vi "Save Profi map Pressure.vi"(0 "Pressure":T2(array[cluster]), 1 "configuration file path":path, 3 "error in":errorcluster, 4 "Write":bool) -> (7 "Array":T2(array[cluster]), 10 "error out":errorcluster)   [LabVIEW 2025]
uses:
  <vilib>/Utility/config.llb/NI_LVConfig.lvlib
  controls/Tempratures.ctl
  controls/Profi address.ctl
  <vilib>/Utility/config.llb/Read Key (String).vi
  <vilib>/Utility/config.llb/Write Key (String).vi
  controls/Power Meters.ctl
panel:
  in  "Power Meters":cluster{"Select Item 3":T1, "Combo Box 2":T3}[](array[cluster])
  in  "Tempratures":cluster{"Sensor":T4, "Profi":T1}[][](array[cluster])
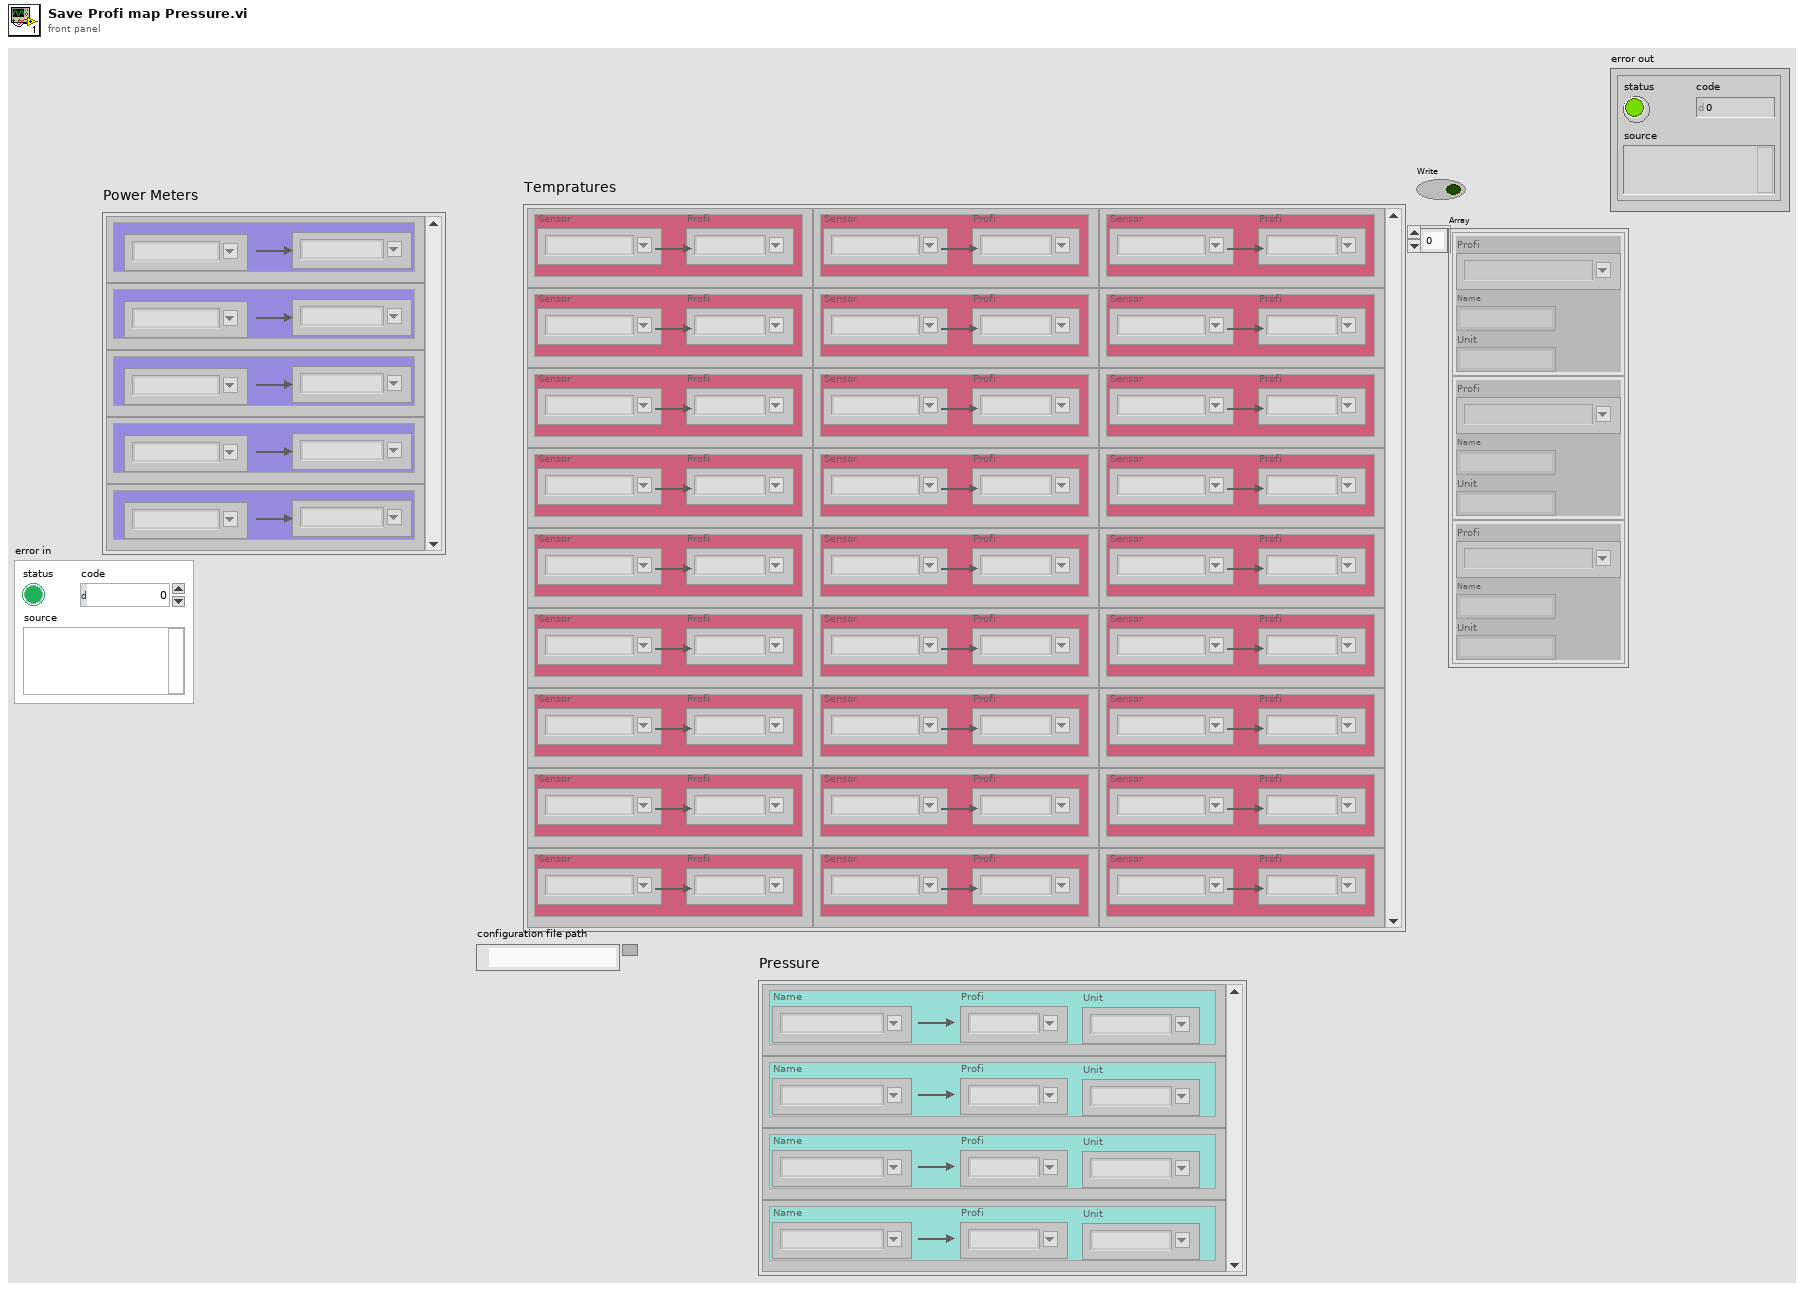
[diagram p1: front panel]
types:
  T1 = typedef "Profi address.ctl" = string
  T2 = cluster{"Profi":T1, "Name":string, "Unit":string}[]
  T3 = typedef "Power Meters.ctl" = string
  T4 = typedef "Tempratures.ctl" = string
  T5 = cluster{"Profi":T1, "Name":string, "Unit":string}
  T6 = typedef "NI_LVConfig.lvlib/Config Data RefNum.ctl" = refnum<k1>
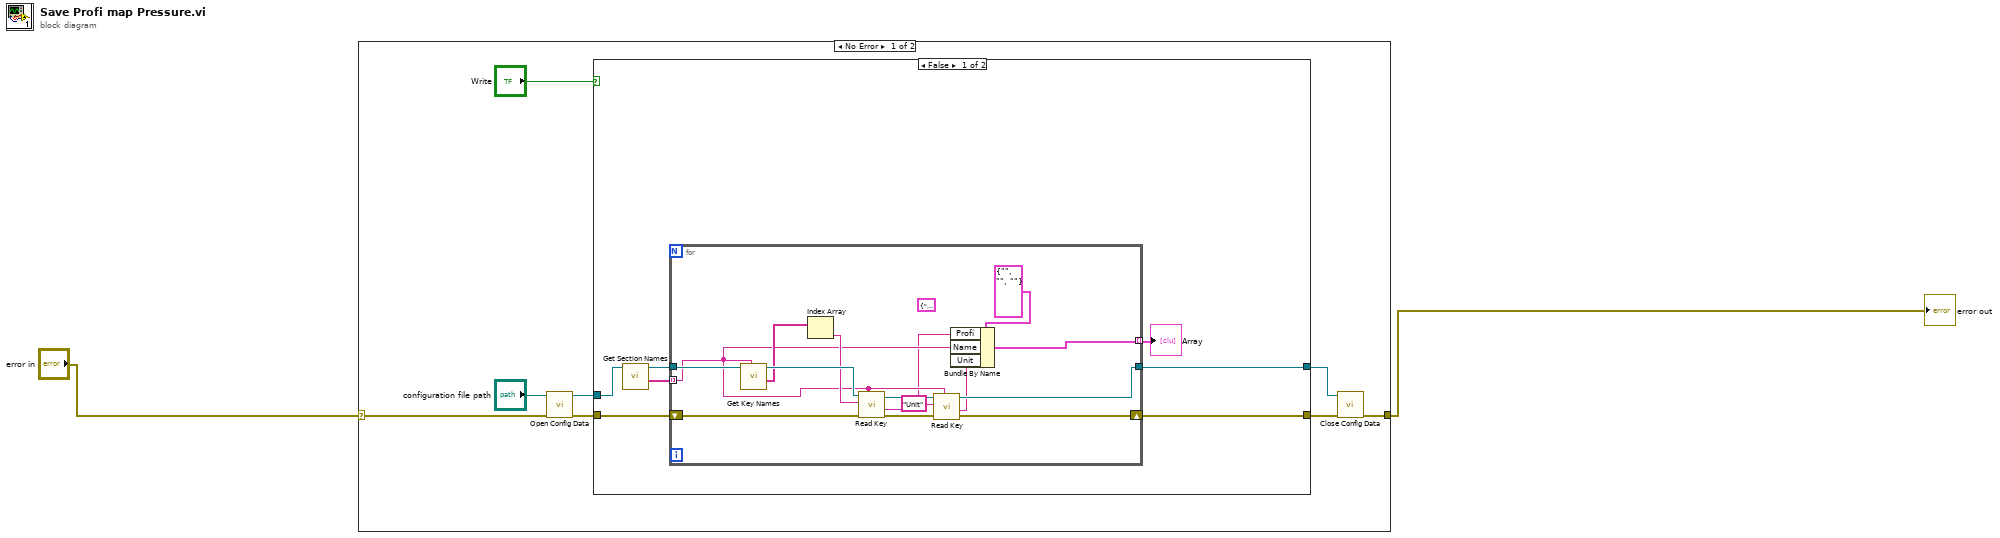
[diagram p0: block diagram]
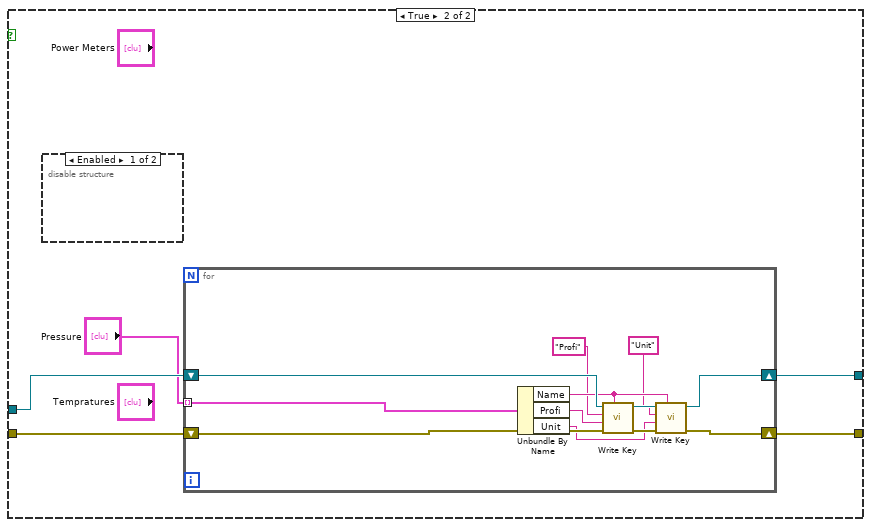
[diagram p2: hidden frame]
diagram:
  n1 = case shown="No Error" "error in" {
    selector: "error in" -> [w5 w49]
    tunnel: [w6 w49] -> w1
    frame No Error {
      n2 = call <vilib>:"Open Config Data.vi"("error in (no error)"=w5, "configuration file path"="configuration file path") -> ("error out"=w4:errorcluster, "refnum"=w10:T6)  [unwired: 7 in, 1 out]
      n3 = case shown="False" "Write" {
        tunnel: w10 -> [w16 w36]
        tunnel: [w17 w35] -> w7
        tunnel: w4 -> [w13 w34]
        tunnel: [w12 w33] -> w3
        frame False {
          n4 = call <vilib>:"Get Section Names.vi"("refnum"=w16) -> ("section names"=w15:string[], "refnum out"=w14:T6)  [unwired: 8 in, 1 out]
          n5 = for {
            tunnel: [w22] -> w17
            tunnel: w15 -> [w19] mode=indexing
            tunnel: w14 -> [w30]
            tunnel: [w29] -> w11 mode=indexing
            shift-right: [w27] -> w12
            shift-left: w13 -> [w28]
            (unwired) cluster{"Sensor":T4, "Profi":T1} {"Sensor"="", "Profi"=""} ("Cluster 6")
            n6 = call <vilib>:"Get Key Names.vi"("section"=w19, "refnum"=w30) -> ("key names"=w26:string[], "refnum out"=w31:T6)  [unwired: 6 in, 2 out]
            n7 = Index Array(array=w26) -> (element=w25:string)  [unwired: 1 in]
            n8 = call-poly <vilib>:"Read Key.vi"("section"=w19, "error in (no error)"=w28, "key"=w25, "refnum"=w31) -> ("error out"=w27:errorcluster, "value"=w18:string, "refnum out"=w23:T6)  [unwired: 4 in, 1 out]
            n9 = call-poly <vilib>:"Read Key.vi"("section"=w19, "key"="Unit", "refnum"=w23) -> ("value"=w20:string, "refnum out"=w22:T6)  [unwired: 5 in, 2 out]
            n10 = Bundle By Name(cluster=T5 {"Profi"="", "Name"="", "Unit"=""} ("Cluster 8"), "Profi"=w18, "Name"=w19, "Unit"=w20) -> (w29:T5)
          }
          "Array" <- w11
        }
        frame True {
          n11 = disable-structure shown="Enabled" {
            frame Enabled {
            }
            frame Disabled {
            }
          }
          n12 = for {
            tunnel: "Pressure" -> [w48] mode=indexing
            shift-right: [w46] -> w35
            shift-left: w36 -> [w47]
            shift-right: [w44] -> w33
            shift-left: w34 -> [w45]
            n13 = Unbundle By Name(w48) -> ("Name"=w41:string, "Profi"=w38:T1, "Unit"=w37:string)
            n14 = call-poly <vilib>:"Write Key.vi"("section"=w41, "error in (no error)"=w45, "value"=w38, "key"="Profi", "refnum"=w47) -> ("error out"=w42:errorcluster, "refnum out"=w43:T6)  [unwired: 4 in, 1 out]
            n15 = call-poly <vilib>:"Write Key.vi"("section"=w41, "error in (no error)"=w42, "value"=w37, "key"="Unit", "refnum"=w43) -> ("error out"=w44:errorcluster, "refnum out"=w46:T6)  [unwired: 4 in, 1 out]
          }
        }
      }
      n16 = call <vilib>:"Close Config Data.vi"("error in (no error)"=w3, "refnum"=w7) -> ("error out"=w6:errorcluster)  [unwired: 8 in, 1 out]
    }
    frame Error {
    }
  }
  "error out" <- w1
